vi "pass_and_fail.vi"() -> ()   [LabVIEW 2018]
panel:
  out "Boolean":bool
  out "PASS/FAIL":string
  in  "Numeric":dbl
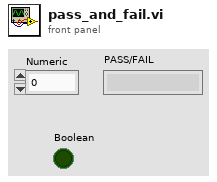
[diagram p1: front panel]
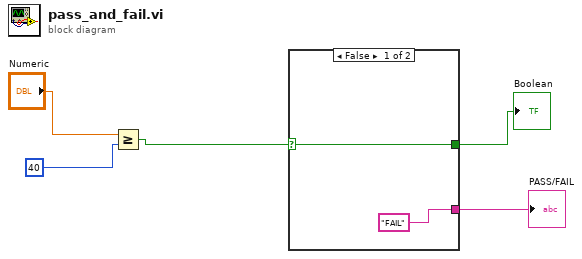
[diagram p0: block diagram]
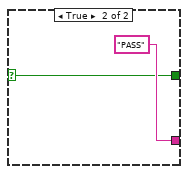
[diagram p2: hidden frame]
diagram:
  n1 = Greater Or Equal?(x="Numeric", y=40) -> (x >= y?=w3:bool)
  n2 = case shown="False" w3 {
    selector: w3 -> [w6 w8]
    tunnel: ["FAIL" "PASS"] -> w2
    tunnel: [w6 w8] -> w1
    frame False {
    }
    frame True {
    }
  }
  "Boolean" <- w1
  "PASS/FAIL" <- w2
